vi "SMU_generateWfm_SaveToText_.vi"() -> ()   [LabVIEW 2025]
uses:
  <vilib>/Utility/file.llb/Write Delimited Spreadsheet (DBL).vi
  <vilib>/measure/NI_MABase.lvlib
panel:
  in  "file path (dialog if empty)":path
  out "Waveform Graph":waveform(dbl)(graph)={"t0"=timestamp(0 s since 1904-01-01), "dt"=1.25e-05, "Y"=[]}
  in  "Square wave duty cycle (%)":dbl=50.0 format="%0.2f"
  in  "Number of Cycles":i32=10
  in  "Amplitude (V)":dbl=1.0 format="%0.2p"
  in  "Frequency (Hz)":dbl=1000.0 format="%0.2p"
  in  "Signal Type":T1(ring)
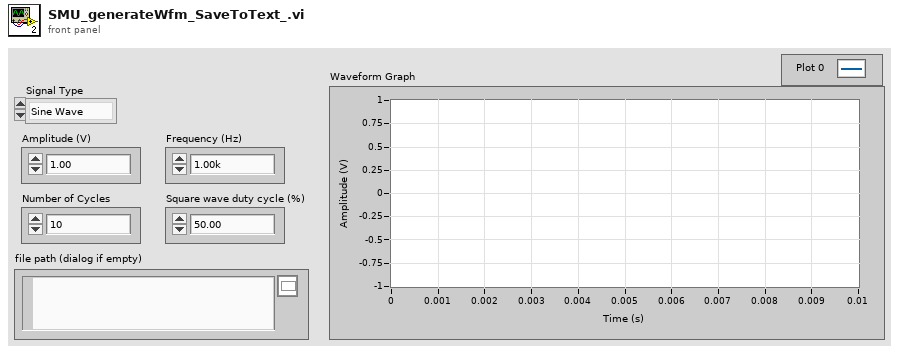
[diagram p1: front panel]
types:
  T1 = enum16{"Sine Wave", "Triangle Wave", "Square Wave", "Sawtooth Wave"}
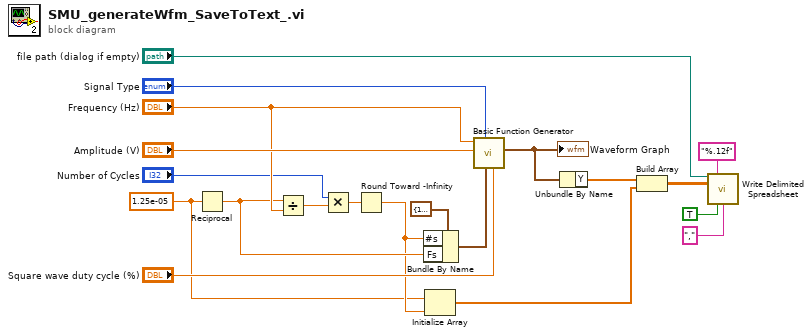
[diagram p0: block diagram]
diagram:
  w2 = 1.25e-05 ("x")
  n1 = Reciprocal(x=w2) -> (1/x=w14:dbl)
  n2 = Divide(x=w14, y="Frequency (Hz)") -> (x/y=w13:dbl)
  n3 = Multiply(x="Number of Cycles", y=w13) -> (x*y=w11:dbl)
  n4 = Round Toward -Infinity(1:w11) -> (0:w3:dbl)
  n5 = Bundle By Name(cluster=cluster{"Fs":dbl, "#s":dbl} {"Fs"=1000.0, "#s"=1000.0} ("sampling info"), "#s"=w3, "Fs"=w14) -> (w16:cluster{"Fs":dbl, "#s":dbl})
  n6 = Initialize Array(w2, w3) -> (w1:dbl[])
  n7 = call <vilib>:"Basic Function Generator.vi"("square wave duty cycle (%)"="Square wave duty cycle (%)", "sampling info"=w16, "signal type"="Signal Type", "amplitude"="Amplitude (V)", "frequency"="Frequency (Hz)") -> ("signal out"=w10:waveform(dbl))  [unwired: 4 in, 2 out]
  "Waveform Graph" <- w10
  n8 = Unbundle By Name(w10) -> ("Y"=w9:dbl[])
  n9 = Build Array(w9, w1) -> (w8:dbl[][])
  n10 = call-poly <vilib>:"Write Delimited Spreadsheet.vi"("file path (dialog if empty)"="file path (dialog if empty)", "format (%.3f)"="%.12f", "2D data"=w8, "transpose? (no:F)"=TRUE, "delimiter (\\t)"="," ("delimiter (\\t)")) -> ()  [unwired: 9 in, 2 out]
